vi "Create-Destroy.vi"(5 "Username":string, 6 "Password":string, 7 "Address":string, 8 "Error In":errorcluster) -> (0 "Error Out":errorcluster)   [LabVIEW 2018, in "Tests.lvlib" / "SFTP.lvlib"]
uses:
  SFTP.lvlib
  src/Toolkit/SFTP/Support/Create from Session.vi
  src/Toolkit/SFTP/Support/Destroy to Session.vi
  <vilib>/addons/_JKI Toolkits/Caraya/classes/Test/Test.lvclass
  <vilib>/addons/_JKI Toolkits/Caraya/classes/Assert/Assert.lvclass
  src/Toolkit/SFTP/SFTP.lvclass
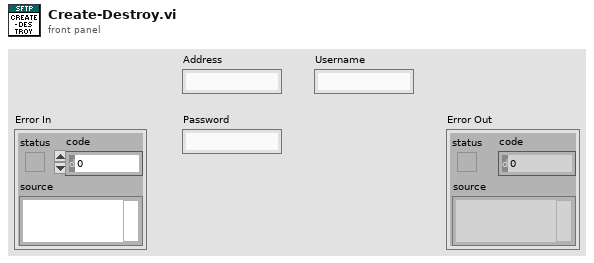
[diagram p1: front panel]
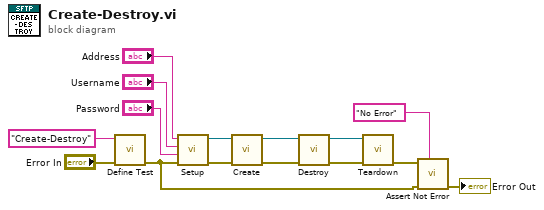
[diagram p0: block diagram]
diagram:
  n1 = call <vilib>:"Define Test.vi"("error in (no error)"="Error In", "Label (VI Title)"="Create-Destroy") -> ("error out"=w9:errorcluster)  [unwired: 9 in]
  n2 = call "Setup.vi"("Error In"=w9, "Password"="Password", "Username"="Username", "Address"="Address") -> ("Error Out"=w10:errorcluster, "Sesssion"=w5:refnum<class "Session.lvclass">)  [unwired: 6 in]
  n3 = call-poly "Create.vi"("Error In"=w10, "Session"=w5) -> ("Error Out"=w11:errorcluster, "SFTP"=w2:refnum<class "SFTP.lvclass">)  [unwired: 8 in]
  n4 = call-poly "Destroy.vi"("Error In"=w11, "SFTP"=w2) -> ("Error Out"=w4:errorcluster, "Session"=w1:refnum<class "Session.lvclass">)  [unwired: 8 in]
  n5 = call "Teardown.vi"("Error In"=w4, "Session"=w1) -> ("Error Out"=w3:errorcluster)  [unwired: 9 in]
  n6 = call <vilib>:"Assert Not Error.vi"("Label"="No Error", "error in (no error)"=w9, "Not Error?"=w3) -> ("error out"=→"Error Out":errorcluster)  [unwired: 8 in]
